vi "Make Output Property Schema.vi"(8 "error in":errorcluster, 10 "terminals":T1(array[cluster]), 11 "output":T2) -> (0 "error out":errorcluster, 2 "listed?":bool, 3 "property schema":string)   [LabVIEW 2020, in "MCP Server.lvlib"]
doc: "Makes the outputSchema property of one output of a tool, for Make Output Schema.vi: the type schema of the indicator (sub type of its terminal) merged over its MCP type and description, without default. listed? is false for a picture output and for an output without a terminal, which outputSchema leaves out."
uses:
  MCP Server.lvlib
  0c7a5f67-d265-4f18-ab55-abe1618fe39f.vi
  1886bae2-f85c-4b44-ba4a-dea72d5b33b1.vi
  <vilib>/JDP Science/JSONtext/Variant to JSON Text.vi
  <vilib>/JDP Science/JSONtext/support/Format JSON Object.vi
  <vilib>/JDP Science/JSONtext/Set Multiple Object Items.vi
  <vilib>/JDP Science/JSONtext/LVClass Serializer/JSONtext LVClass Serializer.lvclass
  <vilib>/JDP Science/JSONtext/JSONtext.lvlib
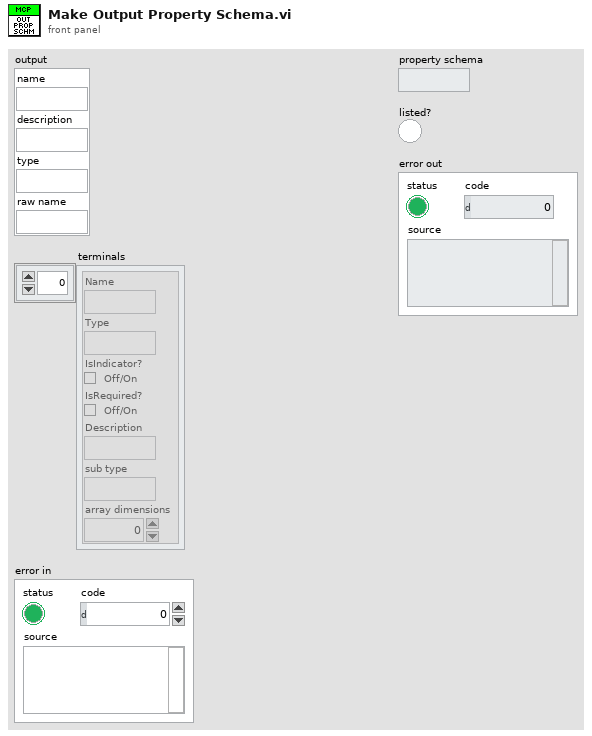
[diagram p1: front panel]
types:
  T1 = cluster{"Name":string, "Type":string, "IsIndicator?":bool, "IsRequired?":bool, "Description":string, "sub type":string, "array dimensions":i32}[]
  T2 = cluster{"name":string, "description":string, "type":string, "raw name":string}
  T3 = cluster{"Name":string, "Type":string, "IsIndicator?":bool, "IsRequired?":bool, "Description":string, "sub type":string, "array dimensions":i32}
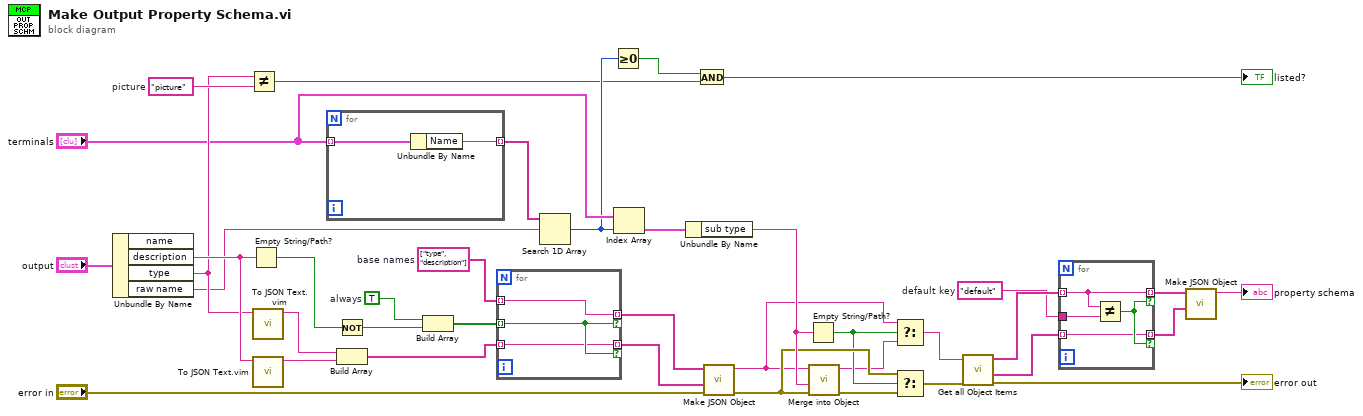
[diagram p0: block diagram]
diagram:
  w27 = TRUE  # always
  w6 = "default"  # default key
  w22 = string[] ["type", "description"]  # base names
  w36 = "picture"  # picture
  n1 = Unbundle By Name("output") -> ("description"=w37:string, "type"=w35:string, "raw name"=w33:string)  [unwired: 1 out]
  n2 = Not Equal?(x=w35, y=w36) -> (x != y?=w23:bool)
  n3 = Empty String/Path?(string/path=w37) -> (empty?=w32:bool)
  n4 = call "To JSON Text.vim"("Anything"=w35) -> ("<JSON>"=w31:string)  [unwired: 9 in, 1 out]
  n5 = call "To JSON Text.vim"("Anything"=w37) -> ("<JSON>"=w30:string)  [unwired: 9 in, 1 out]
  n6 = for {
    tunnel: "terminals" -> [w40] mode=indexing
    tunnel: [w39] -> w34 mode=indexing
    n7 = Unbundle By Name(w40) -> ("Name"=w39:string)
  }
  n8 = Not(x=w32) -> (.not. x?=w26:bool)
  n9 = Build Array(w31, w30) -> (w21:string[])
  n10 = Build Array(w27, w26) -> (w20:bool[])
  n11 = for {
    tunnel: w22 -> [w43] mode=indexing
    tunnel: w21 -> [w41] mode=indexing
    tunnel: w20 -> [w42] mode=indexing
    tunnel: [w43] -> w19 mode=indexing if=w42
    tunnel: [w41] -> w18 mode=indexing if=w42
  }
  n12 = Search 1D Array(1D array=w34, element=w33) -> (index of element=w28:i32)  [unwired: 1 in]
  n13 = Greater Or Equal To 0?(x=w28) -> (x >= 0?=w24:bool)
  n14 = Index Array(array="terminals", index=w28) -> (element=w25:T3)
  n15 = Unbundle By Name(w25) -> ("sub type"=w16:string)
  n16 = And(x=w24, y=w23) -> (x .and. y?=→"listed?":bool)
  n17 = call <vilib>:"Make JSON Object.vi"("error in (no error)"="error in", "JSON Items"=w18, "Item Names"=w19) -> ("error out"=w15:errorcluster, "<JSON>"=w13:string)  [unwired: 7 in]
  n18 = Empty String/Path?(string/path=w16) -> (empty?=w12:bool)
  n19 = call <vilib>:"Merge into Object.vi"("error in (no error)"=w15, "JSON Object to Merge"=w16, "JSON"=w13) -> ("error out"=w14:errorcluster, "<JSON>"=w11:string)  [unwired: 6 in]
  n20 = Select(t=w13, s=w12, f=w11) -> (s? t:f=w10:string)
  n21 = Select(t=w15, s=w12, f=w14) -> (s? t:f=w9:errorcluster)
  n22 = call <vilib>:"Get all Object Items.vi"("error in (no error)"=w9, "JSON"=w10) -> ("error out"=→"error out":errorcluster, "<JSON>"=w7:string[], "Item Names"=w8:string[])  [unwired: 6 in, 1 out]
  n23 = for {
    tunnel: w8 -> [w46] mode=indexing
    tunnel: w7 -> [w44] mode=indexing
    tunnel: w6 -> [w47]
    tunnel: [w46] -> w5 mode=indexing if=w45
    tunnel: [w44] -> w4 mode=indexing if=w45
    n24 = Not Equal?(x=w46, y=w47) -> (x != y?=w45:bool)
  }
  n25 = call <vilib>:"Make JSON Object.vi"("JSON Items"=w4, "Item Names"=w5) -> ("<JSON>"=→"property schema":string)  [unwired: 8 in, 1 out]
